vi "edge_finder.vi"(7 "roi_reset":dbl, 8 "pre_mid_far_edge":i32, 9 "pre_mid_near_edge":i32, 10 "current_mid_far_location":cluster{"X":sgl, "Y":sgl}[](array[cluster])=[{"X"=409.1842, "Y"=210.0}, {"X"=440.92856, "Y"=210.0}], 11 "current_mid_near_location":cluster{"X":sgl, "Y":sgl}[](array[cluster])=[{"X"=87.92308, "Y"=210.0}, {"X"=125.36667, "Y"=210.0}]) -> (0 "mid_far_edge":i32, 1 "mid_near_edge":i32, 2 "mid_far_roi_dead":bool, 3 "mid_near_roi_dead":bool)   [LabVIEW 2024]
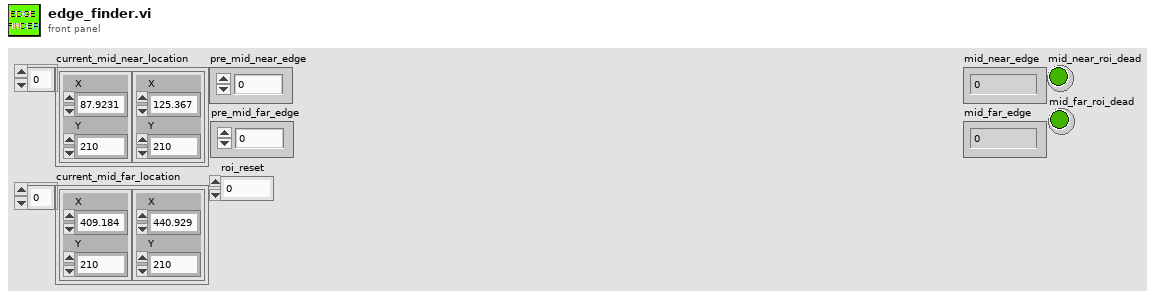
[diagram p1: front panel]
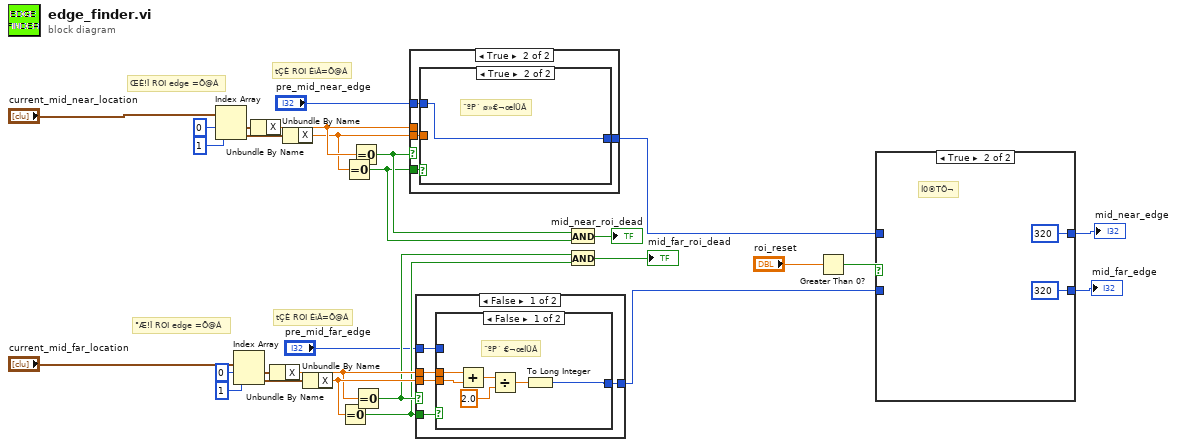
[diagram p0: block diagram]
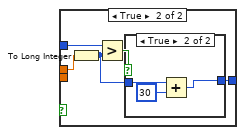
[diagram p3: hidden frame]
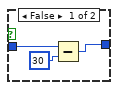
[diagram p4: hidden frame]
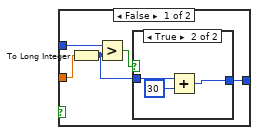
[diagram p6: hidden frame]
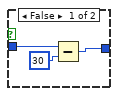
[diagram p7: hidden frame]
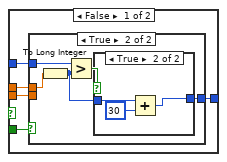
[diagram p8: hidden frame]
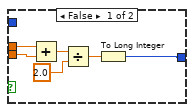
[diagram p9: hidden frame]
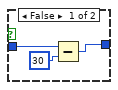
[diagram p10: hidden frame]
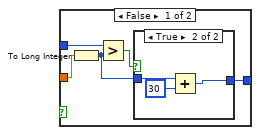
[diagram p11: hidden frame]
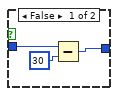
[diagram p12: hidden frame]
diagram:
  # "tÇÈ ROI ÉìÂ=Õ@Á"
  # "tÇÈ ROI ÉìÂ=Õ@Á"
  # "°Æ!Î ROI edge =Õ@Á"
  # "ŒÈ!Î ROI edge =Õ@Á"
  n1 = Index Array(array="current_mid_near_location", index #1=0 ("인덱스"), index #2=1 ("인덱스")) -> (element #1=w24:cluster{"X":sgl, "Y":sgl}, element #2=w23:cluster{"X":sgl, "Y":sgl})
  n2 = Index Array(array="current_mid_far_location", index #1=0 ("인덱스"), index #2=1 ("인덱스")) -> (element #1=w22:cluster{"X":sgl, "Y":sgl}, element #2=w21:cluster{"X":sgl, "Y":sgl})
  n3 = Unbundle By Name(w24) -> ("X"=w16:sgl)
  n4 = Unbundle By Name(w22) -> ("X"=w17:sgl)
  n5 = Unbundle By Name(w23) -> ("X"=w15:sgl)
  n6 = Unbundle By Name(w21) -> ("X"=w20:sgl)
  n7 = Equal To 0?(x=w20) -> (x = 0?=w11:bool)
  n8 = Equal To 0?(x=w15) -> (x = 0?=w13:bool)
  n9 = Equal To 0?(x=w16) -> (x = 0?=w14:bool)
  n10 = Equal To 0?(x=w17) -> (x = 0?=w12:bool)
  n11 = case shown="True" w14 {
    tunnel: w13 -> [w33 w54]
    tunnel: w16 -> [w32 _]
    tunnel: w15 -> [w31 w51]
    tunnel: "pre_mid_near_edge" -> [w29 w53]
    tunnel: [w30 w52] -> w2
    frame False {
      n12 = case shown="True" w33 {
        tunnel: w32 -> [w39 w42]
        tunnel: w31 -> [w38 _]
        tunnel: [w34 w40] -> w30
        tunnel: w29 -> [_ w44]
        frame False {
          n13 = Add(x=w39, y=w38) -> (x+y=w37:sgl)
          n14 = Divide(x=w37, y=sgl 2.0) -> (x/y=w35:sgl)
          n15 = To Long Integer(number=w35) -> (32bit integer=w34:i32)
        }
        frame True {
          n16 = To Long Integer(number=w42) -> (32bit integer=w41:i32)
          n17 = Greater?(x=w44, y=w41) -> (0:w43:bool)
          n18 = case shown="True" w43 {
            tunnel: w41 -> [w47 w50]
            tunnel: [w45 w48] -> w40
            frame False {
              n19 = Subtract(x=w47, y=30) -> (x-y=w45:i32)
            }
            frame True {
              n20 = Add(x=w50, y=30) -> (x+y=w48:i32)
            }
          }
        }
      }
    }
    frame True {
      n21 = case shown="True" w54 {
        tunnel: w53 -> [w59 w66]
        tunnel: [w55 w66] -> w52
        tunnel: w51 -> [w58 _]
        frame False {
          n22 = To Long Integer(number=w58) -> (32bit integer=w56:i32)
          n23 = Greater?(x=w59, y=w56) -> (0:w57:bool)
          n24 = case shown="True" w57 {
            tunnel: [w61 w64] -> w55
            tunnel: w56 -> [w60 w63]
            frame False {
              n25 = Subtract(x=w60, y=30) -> (x-y=w61:i32)
            }
            frame True {
              n26 = Add(x=w63, y=30) -> (x+y=w64:i32)
            }
          }
        }
        frame True {
          # "¨ºP´ ø»€¬œÍÜÂ"
        }
      }
    }
  }
  n27 = case shown="False" w12 {
    tunnel: w11 -> [w71 w92]
    tunnel: w17 -> [w70 _]
    tunnel: w20 -> [w69 w89]
    tunnel: "pre_mid_far_edge" -> [w67 w91]
    tunnel: [w68 w90] -> w1
    frame False {
      n28 = case shown="False" w71 {
        tunnel: w70 -> [w77 w80]
        tunnel: w69 -> [w76 _]
        tunnel: [w72 w78] -> w68
        tunnel: w67 -> [_ w82]
        frame False {
          # "¨ºP´ €¬œÍÜÂ"
          n29 = Add(x=w77, y=w76) -> (x+y=w75:sgl)
          n30 = Divide(x=w75, y=sgl 2.0) -> (x/y=w73:sgl)
          n31 = To Long Integer(number=w73) -> (32bit integer=w72:i32)
        }
        frame True {
          n32 = To Long Integer(number=w80) -> (32bit integer=w79:i32)
          n33 = Greater?(x=w82, y=w79) -> (0:w81:bool)
          n34 = case shown="True" w81 {
            tunnel: w79 -> [w85 w88]
            tunnel: [w83 w86] -> w78
            frame False {
              n35 = Subtract(x=w85, y=30) -> (x-y=w83:i32)
            }
            frame True {
              n36 = Add(x=w88, y=30) -> (x+y=w86:i32)
            }
          }
        }
      }
    }
    frame True {
      n37 = case shown="True" w92 {
        tunnel: w91 -> [w97 w104]
        tunnel: [w93 w104] -> w90
        tunnel: w89 -> [w96 _]
        frame False {
          n38 = To Long Integer(number=w96) -> (32bit integer=w94:i32)
          n39 = Greater?(x=w97, y=w94) -> (0:w95:bool)
          n40 = case shown="True" w95 {
            tunnel: [w99 w102] -> w93
            tunnel: w94 -> [w98 w101]
            frame False {
              n41 = Subtract(x=w98, y=30) -> (x-y=w99:i32)
            }
            frame True {
              n42 = Add(x=w101, y=30) -> (x+y=w102:i32)
            }
          }
        }
        frame True {
        }
      }
    }
  }
  n43 = And(x=w14, y=w13) -> (x .and. y?=→"mid_near_roi_dead":bool)
  n44 = And(x=w12, y=w11) -> (x .and. y?=→"mid_far_roi_dead":bool)
  n45 = Greater Than 0?(x="roi_reset") -> (x > 0?=w5:bool)
  n46 = case shown="True" w5 {
    tunnel: w1 -> [w106 _]
    tunnel: [w106 320 ("상위 리미트")] -> w4
    tunnel: w2 -> [w105 _]
    tunnel: [w105 320 ("하위 리미트")] -> w3
    frame False {
    }
    frame True {
      # "Í0®TÖ¬"
    }
  }
  "mid_near_edge" <- w3
  "mid_far_edge" <- w4
